vi "Tree Filter.vi"(7 "Boolean Connectors":string[](array[string]), 8 "error in":errorcluster, 9 "Comparators":T2(array[cluster]), 10 "Headers":string[](array[string]), 11 "Frame groups":T1(array[cluster])) -> (0 "error out":errorcluster, 1 "Has child field?":bool, 3 "Filtered tree":string[][](array[string]))   [LabVIEW 2025, in "CAN-LIN Raw Bus Capture UI.lvlib"]
uses:
  CAN-LIN Raw Bus Capture UI.lvlib
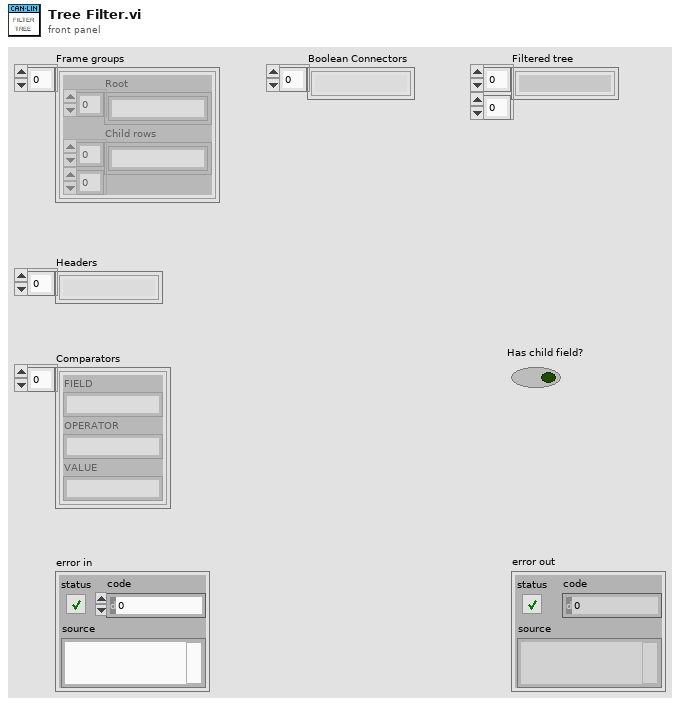
[diagram p1: front panel]
types:
  T1 = cluster{"Root":string[], "Child rows":string[][]}[]
  T2 = cluster{"FIELD":string, "OPERATOR":string, "VALUE":string}[]
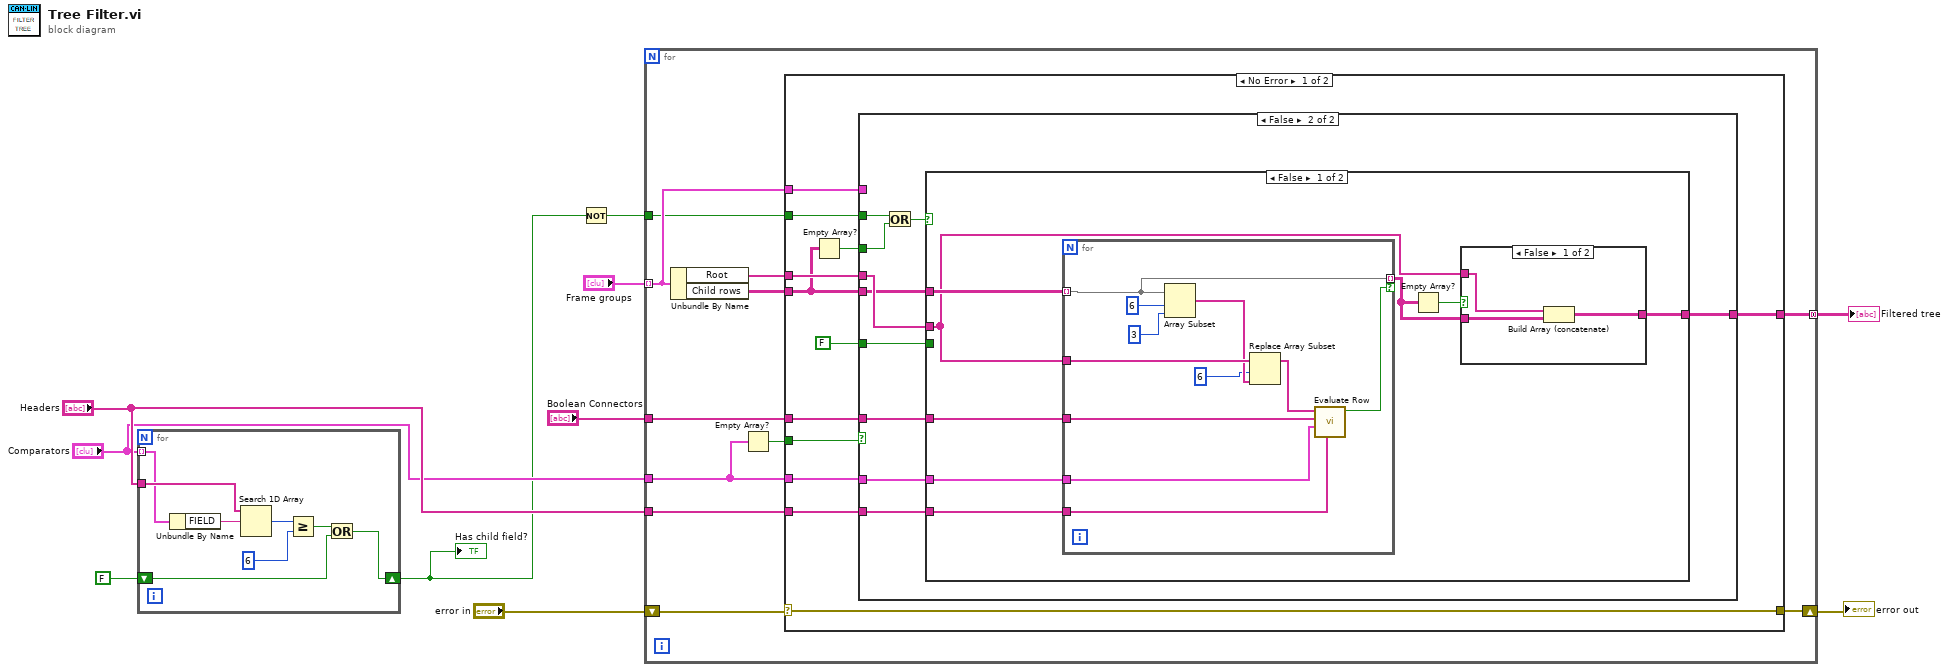
[diagram p0: block diagram]
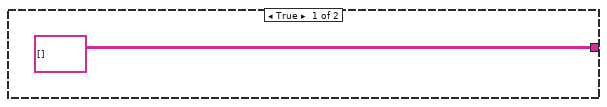
[diagram p2: hidden frame]
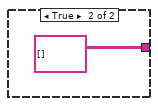
[diagram p3: hidden frame]
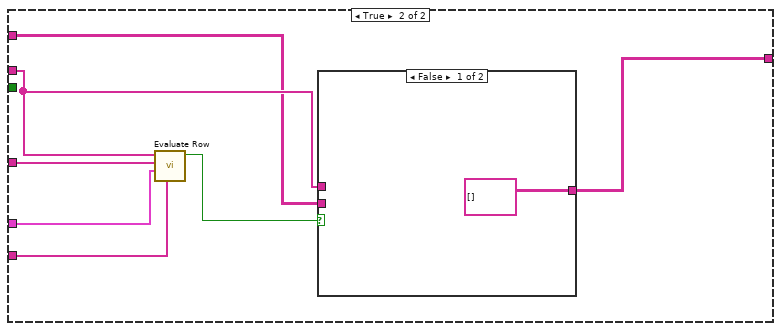
[diagram p4: hidden frame]
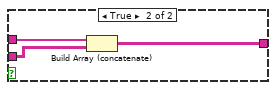
[diagram p5: hidden frame]
diagram:
  n1 = for {
    tunnel: "Headers" -> [w12]
    tunnel: "Comparators" -> [w11] mode=indexing
    shift-right: [w13] -> w2
    shift-left: FALSE ("Has child field?") -> [w14]
    n2 = Unbundle By Name(w11) -> ("FIELD"=w18:string)
    n3 = Search 1D Array(1D array=w12, element=w18) -> (index of element=w17:i32)  [unwired: 1 in]
    n4 = Greater Or Equal?(x=w17, y=6) -> (x >= y?=w15:bool)
    n5 = Or(x=w15, y=w14) -> (x .or. y?=w13:bool)
  }
  "Has child field?" <- w2
  n6 = Not(x=w2) -> (.not. x?=w1:bool)
  n7 = for {
    tunnel: "Frame groups" -> [w24] mode=indexing
    tunnel: "Comparators" -> [w20]
    tunnel: "Boolean Connectors" -> [w29]
    tunnel: "Headers" -> [w27]
    tunnel: [w25] -> w9 mode=concatenating
    shift-right: [w23] -> w8
    shift-left: "error in" -> [w22]
    tunnel: w1 -> [w19]
    n8 = Unbundle By Name(w24) -> ("Root"=w26:string[], "Child rows"=w28:string[][])
    n9 = Empty Array?(array=w20) -> (empty?=w21:bool)
    n10 = case shown="No Error" w22 {
      selector: w22 -> [w38 w87]
      tunnel: w27 -> [w41 _]
      tunnel: w29 -> [w40 _]
      tunnel: w20 -> [w36 _]
      tunnel: w28 -> [w31 _]
      tunnel: [w39 _] -> w25
      tunnel: [w38 w87] -> w23
      tunnel: w26 -> [w35 _]
      tunnel: w24 -> [w34 _]
      tunnel: w21 -> [w33 _]
      tunnel: w19 -> [w32 _]
      frame No Error {
        n11 = Empty Array?(array=w31) -> (empty?=w30:bool)
        n12 = case shown="False" w33 {
          tunnel: w41 -> [_ w52]
          tunnel: FALSE -> [_ w51]
          tunnel: w40 -> [_ w50]
          tunnel: w36 -> [_ w49]
          tunnel: w31 -> [_ w46]
          tunnel: [string[][] [] ("Child rows") w48] -> w39
          tunnel: w35 -> [_ w47]
          tunnel: w34 -> [_ _]
          tunnel: w32 -> [_ w45]
          tunnel: w30 -> [_ w44]
          frame True {
          }
          frame False {
            n13 = Or(x=w45, y=w44) -> (x .or. y?=w43:bool)
            n14 = case shown="False" w43 {
              tunnel: w52 -> [w57 w79]
              tunnel: w51 -> [_ _]
              tunnel: w50 -> [w59 w81]
              tunnel: w49 -> [w58 w80]
              tunnel: [w53 w82] -> w48
              tunnel: w47 -> [w55 w77]
              tunnel: w46 -> [w60 w76]
              frame False {
                n15 = for {
                  tunnel: w60 -> [w66] mode=indexing
                  tunnel: w55 -> [w73]
                  tunnel: w59 -> [w69]
                  tunnel: w58 -> [w68]
                  tunnel: w57 -> [w67]
                  tunnel: [w66] -> w54 mode=indexing if=w65
                  n16 = Array Subset(array=w66, index=6, length=3) -> (w72:string[])
                  n17 = Replace Array Subset(array=w73, new element=w72, index=6) -> (w70:string[])
                  n18 = call "Evaluate Row.vi"("Headers"=w67, "Comparators"=w68, "Boolean Connectors"=w69, "Row"=w70) -> ("Match?"=w65:bool)  [unwired: 7 in]
                }
                n19 = Empty Array?(array=w54) -> (empty?=w56:bool)
                n20 = case shown="False" w56 {
                  tunnel: w55 -> [w63 _]
                  tunnel: w54 -> [w62 _]
                  tunnel: [w61 string[][] []] -> w53
                  frame False {
                    n21 = Build Array (concatenate)(w63, w62) -> (w61:string[][])
                  }
                  frame True {
                  }
                }
              }
              frame True {
                n22 = call "Evaluate Row.vi"("Headers"=w79, "Comparators"=w80, "Boolean Connectors"=w81, "Row"=w77) -> ("Match?"=w78:bool)  [unwired: 7 in]
                n23 = case shown="False" w78 {
                  tunnel: w77 -> [_ w86]
                  tunnel: [string[][] [] w85] -> w82
                  tunnel: w76 -> [_ w84]
                  frame False {
                  }
                  frame True {
                    n24 = Build Array (concatenate)(w86, w84) -> (w85:string[][])
                  }
                }
              }
            }
          }
        }
      }
      frame Error {
      }
    }
  }
  "Filtered tree" <- w9
  "error out" <- w8
